vi "CheckRemoteControl.vi"(0 "Universal Robot.lvclass in":refnum<class "Universal Robot.lvclass">, 5 "error in (no error)":errorcluster) -> (14 "Universal Robot.lvclass out":refnum<class "Universal Robot.lvclass">, 19 "error out":errorcluster)   [LabVIEW 2019, in "Universal Robot.lvclass"]
uses:
  Universal Robot.lvclass
  Universal Robot.lvclass/Universal Robot.ctl
  Client Interfaces/Dashboard Server/Dashboard Server.lvclass
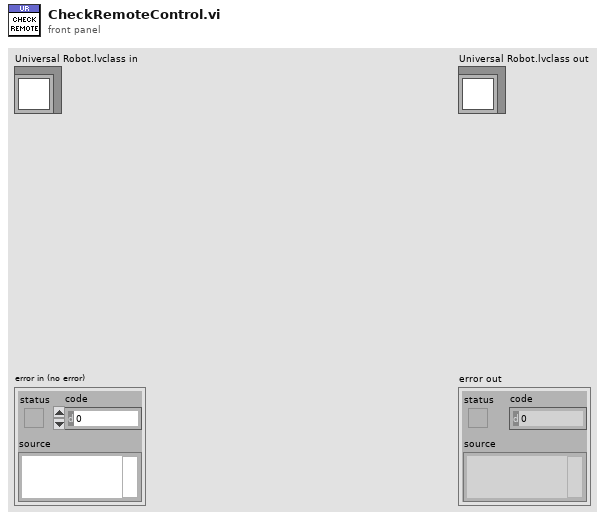
[diagram p1: front panel]
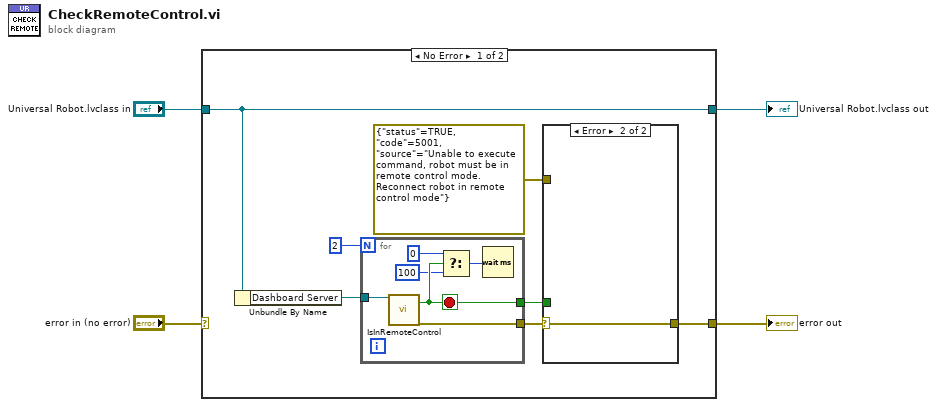
[diagram p0: block diagram]
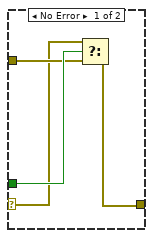
[diagram p2: hidden frame]
diagram:
  n1 = case shown="No Error" "error in (no error)" {
    selector: "error in (no error)" -> [_ w24]
    tunnel: [w8 w24] -> w3
    tunnel: "Universal Robot.lvclass in" -> [w11 w23]
    tunnel: [w11 w23] -> w1
    frame No Error {
      n2 = Unbundle By Name(w11) -> ("Dashboard Server"=w10:refnum<class "Dashboard Server.lvclass">)
      n3 = for {
        N: 2 -> [_]
        tunnel: w10 -> [w17]
        tunnel: [w15] -> w9
        tunnel: [w16] -> w6
        stop <- w15 stop-if-true
        n4 = call-dynamic "IsInRemoteControl.vi"("DashboardServer in"=w17) -> ("remoteControl"=w15:bool, "error out"=w16:errorcluster)  [unwired: 16 in, 1 out]
        n5 = Select(t=u32 0 ("milliseconds to wait"), s=w15, f=u32 100) -> (s? t:f=w13:u32)
        n6 = Wait (ms)(milliseconds to wait=w13) -> ()  [unwired: 1 out]
      }
      n7 = case shown="Error" w6 {
        selector: w6 -> [w18 w22]
        tunnel: w9 -> [w21 _]
        tunnel: [w20 w22] -> w8
        tunnel: errorcluster {"status"=TRUE, "code"=5001, "source"="Unable to execute command, robot must be in remote control mode. Reconnect robot in remote control mode"} ("error constant") -> [w19 _]
        frame No Error {
          n8 = Select(t=w18, s=w21, f=w19) -> (s? t:f=w20:errorcluster)
        }
        frame Error {
        }
      }
    }
    frame Error {
    }
  }
  "error out" <- w3
  "Universal Robot.lvclass out" <- w1
